vi "Write VI Reference.vi"(8 "error in":errorcluster, 10 "VI Reference":refnum<vi>, 11 "LabVIEW File in":refnum<class "LabVIEW File.lvclass">) -> (0 "error out":errorcluster, 3 "LabVIEW File out":refnum<class "LabVIEW File.lvclass">)   [LabVIEW 2026, in "LabVIEW File.lvclass"]
doc: "Data accessor."
uses:
  LabVIEW File.lvclass
  LabVIEW File.lvclass/LabVIEW File.ctl
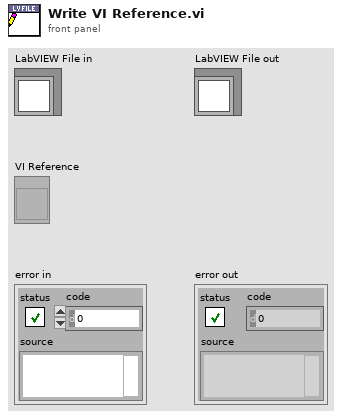
[diagram p1: front panel]
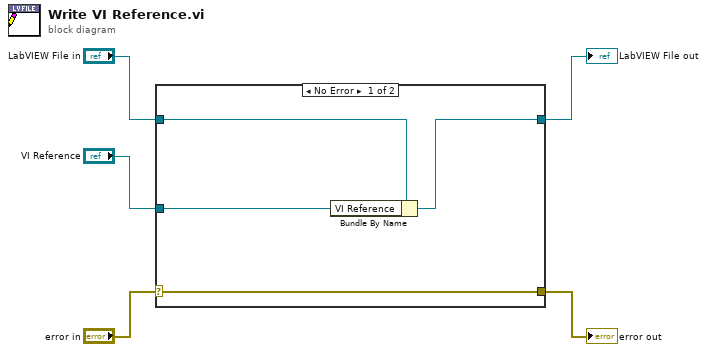
[diagram p0: block diagram]
diagram:
  n1 = case shown="No Error" "error in" {
    selector: "error in" -> [w9 w11]
    tunnel: [w9 w11] -> w4
    tunnel: [w7 w10] -> w2
    tunnel: "LabVIEW File in" -> [w8 w10]
    tunnel: "VI Reference" -> [w6 _]
    frame No Error {
      n2 = Bundle By Name(cluster=w8, "VI Reference"=w6) -> (w7:refnum<class "LabVIEW File.lvclass">)
    }
    frame Error {
      # "Pass error without further action."
    }
  }
  "error out" <- w4
  "LabVIEW File out" <- w2
